vi "easingOut.vi"(8 "d":dbl, 9 "c":dbl, 10 "b":dbl, 11 "t":dbl) -> (3 "return":dbl)   [LabVIEW 2025, in "XButton.lvlib" / "button3.xctl"]
uses:
  button3.xctl
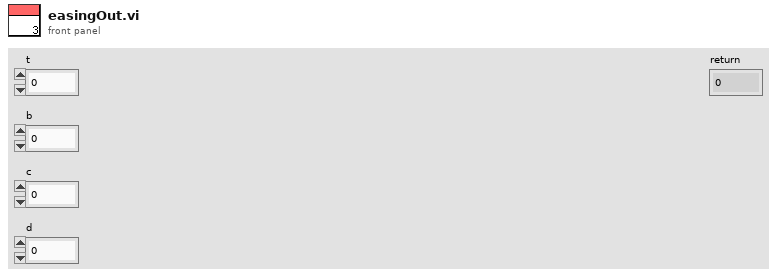
[diagram p1: front panel]
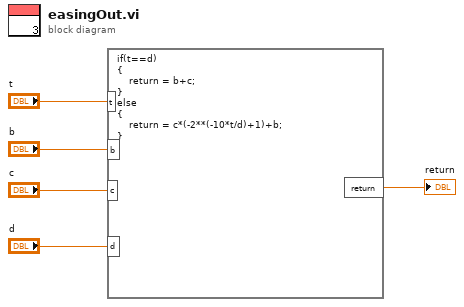
[diagram p0: block diagram]
diagram:
  n1 = formula code="if(t==d)\n{\n    return = b+c;\n}\nelse\n{\n    return = c*(-2**(-10*t/d)+1)+b;\n}"("t"="t", "b"="b", "c"="c", "d"="d") -> ("return"=→"return":dbl)
